vi "FRC Make Dir.vi"(8 "error in":errorcluster, 11 "path":path) -> (0 "error out":errorcluster)   [LabVIEW 2025]
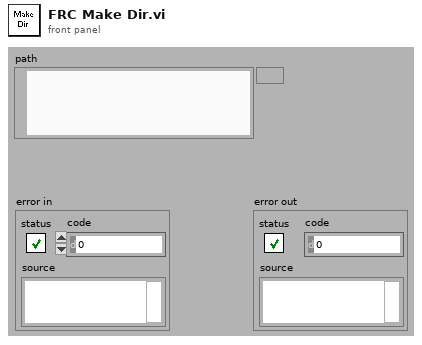
[diagram p1: front panel]
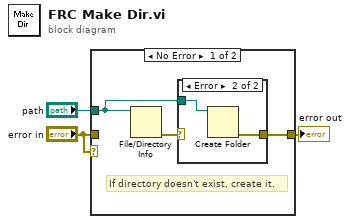
[diagram p0: block diagram]
diagram:
  n1 = case shown="No Error" "error in" {
    tunnel: [w5 w9] -> w3
    tunnel: "error in" -> [_ w9]
    tunnel: "path" -> [w4 _]
    frame No Error {
      # "If directory doesn't exist, create it."
      n2 = File/Directory Info(path=w4) -> (error out=w6:errorcluster)  [unwired: 1 in, 6 out]
      n3 = case shown="Error" w6 {
        tunnel: w4 -> [_ w8]
        tunnel: [_ w7] -> w5
        frame No Error {
        }
        frame Error {
          n4 = Create Folder(path (use dialog)=w8) -> (error out=w7:errorcluster)  [unwired: 1 in, 3 out]
        }
      }
    }
    frame Error {
    }
  }
  "error out" <- w3
